vi "String To Number(U32).vi"(5 "String":string) -> (0 "Numeric(U32)":u32)   [LabVIEW 2017]
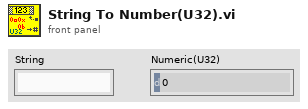
[diagram p1: front panel]
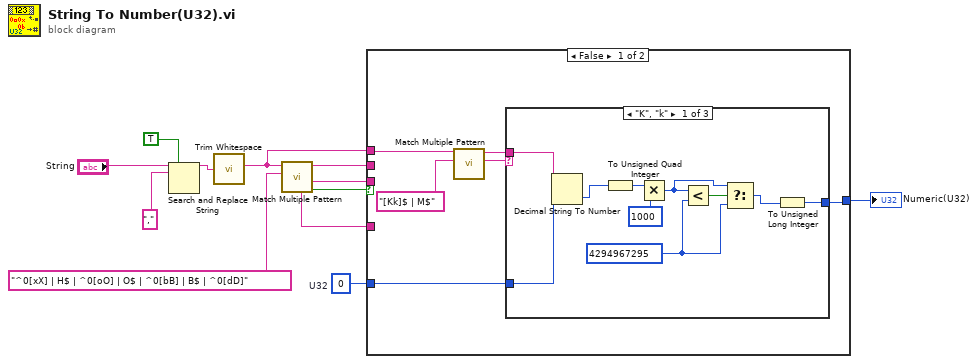
[diagram p0: block diagram]
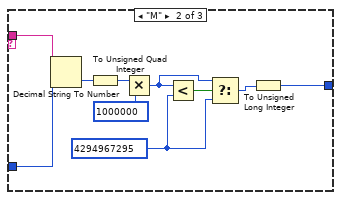
[diagram p2: hidden frame]
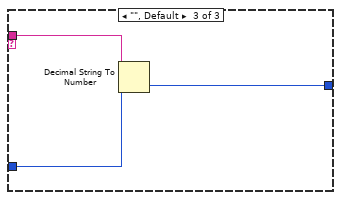
[diagram p3: hidden frame]
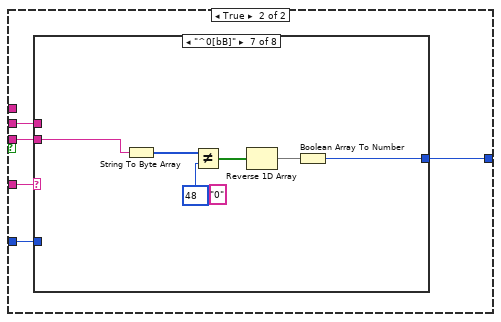
[diagram p4: hidden frame]
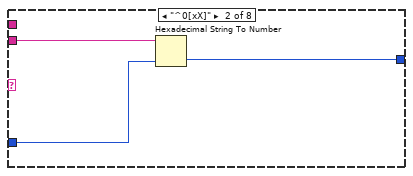
[diagram p6: hidden frame]
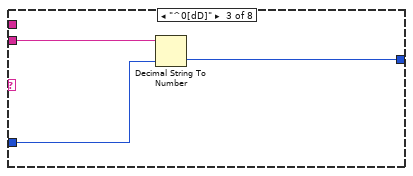
[diagram p7: hidden frame]
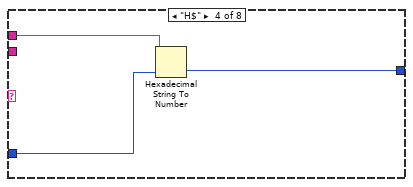
[diagram p8: hidden frame]
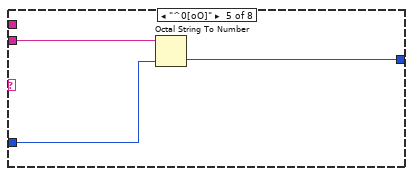
[diagram p9: hidden frame]
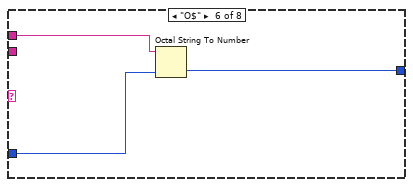
[diagram p10: hidden frame]
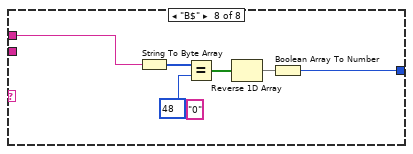
[diagram p11: hidden frame]
diagram:
  w1 = u32 0  # U32
  n1 = Search and Replace String(replace all?=TRUE ("replace all? (F)"), input string="String", search string=",") -> (result string=w9:string)  [unwired: 5 in, 3 out]
  n2 = call <vilib>:"Trim Whitespace.vi"("string"=w9) -> ("trimmed string"=w2:string)  [unwired: 1 in]
  n3 = call "Match Multiple Pattern.vi"("regular expression"="^0[xX] | H$ | ^0[oO] | O$ | ^0[bB] | B$ | ^0[dD]", "string"=w2) -> ("Found?"=w7:bool, "after substring"=w5:string, "before substring"=w4:string, "pattern matched"=w6:string)  [unwired: 5 in, 1 out]
  n4 = case shown="False" w7 {
    tunnel: w6 -> [_ w46]
    tunnel: w5 -> [_ w45]
    tunnel: w4 -> [_ w44]
    tunnel: [w13 w43] -> w3
    tunnel: w2 -> [w15 _]
    tunnel: w1 -> [w14 w42]
    frame False {
      n5 = call "Match Multiple Pattern.vi"("regular expression"="[Kk]$ | M$", "string"=w15) -> ("match substring"=w17:string, "before substring"=w16:string)  [unwired: 5 in, 3 out]
      n6 = case shown="\"K\", \"k\"" w17 {
        tunnel: [w19 w29 w41] -> w13
        tunnel: w14 -> [w27 w37 w40]
        tunnel: w16 -> [w28 w38 w39]
        frame "K", "k" {
          w22 = u32 4294967295 ("y")
          n7 = Decimal String To Number(string=w28, default (0L)=w27) -> (number=w21:u32)  [unwired: 1 in, 1 out]
          n8 = To Unsigned Quad Integer(1:w21) -> (0:w25:u64)
          n9 = Multiply(x=w25, y=u64 1000) -> (x*y=w23:u64)
          n10 = Less?(x=w23, y=w22) -> (x < y?=w24:bool)
          n11 = Select(t=w23, s=w24, f=w22) -> (s? t:f=w20:u64)
          n12 = To Unsigned Long Integer(number=w20) -> (unsigned 32bit integer=w19:u32)
        }
        frame "M" {
          w30 = u32 4294967295 ("y")
          n13 = Decimal String To Number(string=w38, default (0L)=w37) -> (number=w36:u32)  [unwired: 1 in, 1 out]
          n14 = To Unsigned Quad Integer(1:w36) -> (0:w34:u64)
          n15 = Multiply(x=w34, y=u64 1000000) -> (x*y=w32:u64)
          n16 = Less?(x=w32, y=w30) -> (x < y?=w33:bool)
          n17 = Select(t=w32, s=w33, f=w30) -> (s? t:f=w31:u64)
          n18 = To Unsigned Long Integer(number=w31) -> (unsigned 32bit integer=w29:u32)
        }
        frame "", Default {
          n19 = Decimal String To Number(string=w39, default (0L)=w40) -> (number=w41:u32)  [unwired: 1 in, 1 out]
        }
      }
    }
    frame True {
      n20 = case shown="\"^0[bB]\"" w46 {
        tunnel: w45 -> [_ w50 w53 _ w59 _ w67 _]
        tunnel: w44 -> [_ _ _ w55 _ w61 _ w71]
        tunnel: [w47 w49 w52 w56 w58 w62 w68 w74] -> w43
        tunnel: w42 -> [w47 w48 w51 w54 w57 w60 _ _]
        frame Default {
        }
        frame "^0[xX]" {
          n21 = Hexadecimal String To Number(string=w50, default (0uL)=w48) -> (number=w49:u32)  [unwired: 1 in, 1 out]
        }
        frame "^0[dD]" {
          n22 = Decimal String To Number(string=w53, default (0L)=w51) -> (number=w52:u32)  [unwired: 1 in, 1 out]
        }
        frame "H$" {
          n23 = Hexadecimal String To Number(string=w55, default (0uL)=w54) -> (number=w56:u32)  [unwired: 1 in, 1 out]
        }
        frame "^0[oO]" {
          n24 = Octal String To Number(2:w57, 4:w59) -> (0:w58:u32)  [unwired: 1 in, 1 out]
        }
        frame "O$" {
          n25 = Octal String To Number(2:w60, 4:w61) -> (0:w62:u32)  [unwired: 1 in, 1 out]
        }
        frame "^0[bB]" {
          (unwired) "0" ("search string")
          n26 = String To Byte Array(string=w67) -> (unsigned byte array=w66:u8[])
          n27 = Not Equal?(x=w66, y=u8 48) -> (x != y?=w64:bool[])
          n28 = Reverse 1D Array(array=w64) -> (reversed array=w63:bool[])
          n29 = Boolean Array To Number(Boolean array=w63) -> (number=w68:u32)
        }
        frame "B$" {
          (unwired) "0" ("search string")
          n30 = String To Byte Array(string=w71) -> (unsigned byte array=w73:u8[])
          n31 = Equal?(x=w73, y=u8 48) -> (x = y?=w72:bool[])
          n32 = Reverse 1D Array(array=w72) -> (reversed array=w70:bool[])
          n33 = Boolean Array To Number(Boolean array=w70) -> (number=w74:u32)
        }
      }
    }
  }
  "Numeric(U32)" <- w3
